vi "Launch Autocomplete Handler.vi"(4 "Shared Options (Local)":refnum<class "Shared Options.lvclass">, 5 "Autohide ListBox (F)":bool, 6 "Allow Undefined Values (F)":bool, 7 "ListBox Refnum (Popup)":refnum<vi>, 8 "error in (no error)":errorcluster, 9 "Height (200)":i16=200, 10 "Initial Options (Empty)":string[](array[string]), 11 "Str Refnum":refnum<vi>) -> (0 "error out":errorcluster, 1 "New Options Event":refnum<user-event>, 2 "Stop Event":refnum<user-event>, 3 "Selection":refnum<user-event>)   [LabVIEW 2020, in "AutoComplete.lvlib"]
doc: "Creates a standalone AutoComplete handler with separate events for interaction. Register for the <b>Selection</b> event to receive selections made by users with autocomplete. <b>Stop</b> and <b>New Options</b> events are for interacting to the autocomplete handler.\n\n<b>Str Refnum</b> - The control that drives the search functionality and has the result placed in.\n<b>Initial Options</b> - The starting list of possible selections. This can bae updated later by generating a New Options event.\n<b>Height</b> - Sets the pixel height of the popup list when typing into the specified string.\n<b>ListBox Refnum</b> - Alternatively a separate ListBox can be specified that is integrated into the UI.\n<b>Autohide ListBox</b> - When specifying an external ListBox, this causes the listbox to be hidden whenever a selection is made.\n<b>Allow Undefined Values</b> - Allows users to enter arbitrary values in addition to what is available in the options list.\n<b>Shared Options</b> - Uses the Shared Options instance, if valid, to filter available options from. If a Shared Options instance is specified, the Selection event output will not be available for use."
uses:
  AutoComplete.lvlib
  Shared Options/Shared Options.lvclass
  Shared Options/Shared Options.lvclass/Shared Options.ctl
  f473066a-8c46-4ba7-8d54-d92ea80dbf8d.vi/ff40df25-0e41-4205-825d-56c19dc320b6.vi
  <vilib>/Utility/Debug Log/Display.vi
  Autocomplete UI.vi
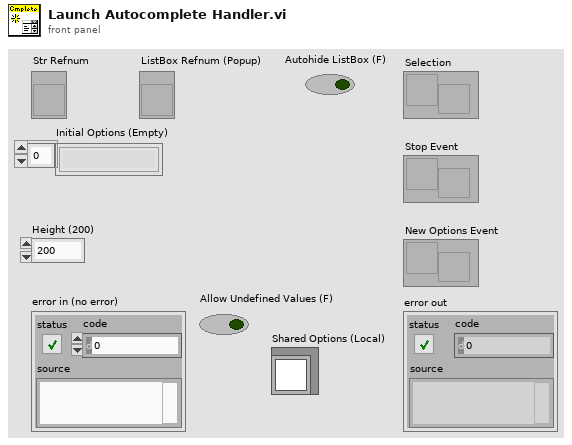
[diagram p1: front panel]
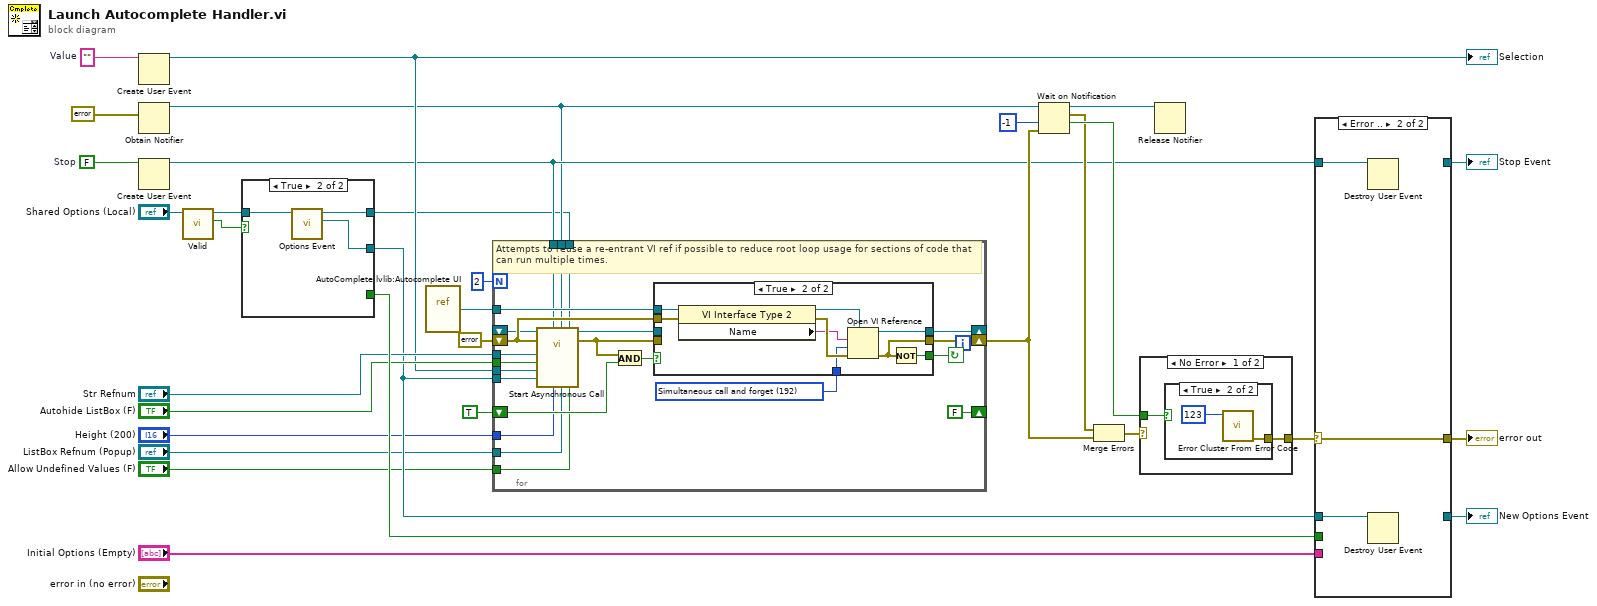
[diagram p0: block diagram]
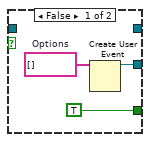
[diagram p3: hidden frame]
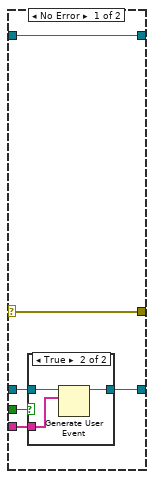
[diagram p6: hidden frame]
diagram:
  w20 = ""  # Value
  w32 = FALSE  # Stop
  n1 = Create User Event(user event datatype=w20) -> (user event=w9:refnum<user-event>)  [unwired: 1 in, 1 out]
  "Selection" <- w9
  n2 = Obtain Notifier(notification data type=errorcluster {"status"=FALSE, "code"=0, "source"=""} ("error constant")) -> (notifier out=w3:refnum<notifier>)  [unwired: 3 in, 2 out]
  n3 = Create User Event(user event datatype=w32) -> (user event=w4:refnum<user-event>)  [unwired: 1 in, 1 out]
  n4 = call "Valid.vi"("Shared Options in"="Shared Options (Local)") -> ("Valid"=w18:bool, "Shared Options out"=w17:refnum<class "Shared Options.lvclass">)  [unwired: 8 in, 1 out]
  n5 = case shown="True" w18 {
    tunnel: w17 -> [_ w38]
    tunnel: [w34 w36] -> w8
    tunnel: [_ w37] -> w2
    tunnel: [TRUE _] -> w16
    frame False {
      w35 = string[] []  # Options
      n6 = Create User Event(user event datatype=w35) -> (user event=w34:refnum<user-event>)  [unwired: 1 in, 1 out]
    }
    frame True {
      n7 = call "Options Event.vi"("Shared Options in"=w38) -> ("Options Event"=w36:refnum<user-event>, "Shared Options out"=w37:refnum<class "Shared Options.lvclass">)  [unwired: 8 in, 1 out]
    }
  }
  n8 = vi-ref "AutoComplete.lvlib:Autocomplete UI.vi"() -> (w14:refnum<vi>)
  n9 = for {
    N: 2 -> [_]
    tunnel: w14 -> [w59]
    shift-right: [w58] -> _
    shift-left: _ -> [w57]
    shift-right: [w55] -> w12
    shift-left: errorcluster {"status"=FALSE, "code"=0, "source"=""} ("error out") -> [w60]
    shift-right: [FALSE] -> _
    shift-left: TRUE -> [w52]
    tunnel: "Str Refnum" -> [w48]
    tunnel: "Autohide ListBox (F)" -> [w47]
    tunnel: w9 -> [w46]
    tunnel: w8 -> [w45]
    tunnel: "Height (200)" -> [w44]
    tunnel: "ListBox Refnum (Popup)" -> [w43]
    tunnel: "Allow Undefined Values (F)" -> [w42]
    tunnel: w4 -> [w41]
    tunnel: w3 -> [w40]
    tunnel: w2 -> [w39]
    stop <- w51 continue-if-true
    w49 = 192 items=["Record modifications"=1, "Open templates for editing"=2, "Prompt user to save"=4, "Prepare for reentrant run"=8, "Prompt to find missing subVIs"=16, "Hide loading dialog box"=32, "Enable simultaneous calls"=64, "Prepare to call and forget"=128, "Simultaneous call and forget"=192, "Prepare to call and collect"=256, "Simultaneous call and collect"=320]
    # "Attempts to reuse a re-entrant VI ref if possible to reduce root loop usage for sections of code that can run multiple times."
    n10 = call-by-ref "Start Asynchronous Call"(reference=w57, error in=w60, "Allow Undefined Values? (F)"=w42, "Shared Options (Local)"=w39, "LstBox Refnum"=w43, "Ready Notifier"=w40, "Height (200)"=w44, "Stop Event"=w41, "Options"=w45, "Selection Event"=w46, "Autohide ListBox (F)"=w47, "Str Refnum"=w48) -> (reference out=w56:refnum<vi>, error out=w54:errorcluster)  [unwired: 2 in]
    n11 = And(x=w54, y=w52) -> (x .and. y?=w53:bool)
    n12 = case shown="True" w53 {
      tunnel: w59 -> [_ w70]
      tunnel: w49 -> [_ w68]
      tunnel: [w62 w66] -> w58
      tunnel: w56 -> [w62 _]
      tunnel: [w61 w64] -> w55
      tunnel: w54 -> [w61 _]
      tunnel: w60 -> [_ w65]
      tunnel: [_ w63] -> w51
      frame False {
      }
      frame True {
        n13 = property class="VI Interface Type 2"(reference=w70, error in=w65) -> (reference out=w67:refnum<vi>, error out=w71:errorcluster, "Name"=w69:string)
        n14 = Open VI Reference(type specifier VI Refnum (for type only)=w67, vi path=w69, options=w68, error in (no error)=w71) -> (vi reference=w66:refnum<vi>, error out=w64:errorcluster)  [unwired: 2 in]
        n15 = Not(x=w64) -> (.not. x?=w63:bool)
      }
    }
  }
  n16 = Wait on Notification(notifier=w3, timeout in ms (-1)=-1, error in (no error)=w12) -> (notifier out=w29:refnum<notifier>, notification=w22:errorcluster, timed out?=w28:bool)  [unwired: 1 in, 1 out]
  n17 = Merge Errors(w22, w12) -> (w21:errorcluster)
  n18 = case shown="No Error" w21 {
    selector: w21 -> [_ w76]
    tunnel: w28 -> [w73 _]
    tunnel: [w72 w76] -> w27
    frame No Error {
      n19 = case shown="True" w73 {
        tunnel: [_ w74] -> w72
        frame False {
        }
        frame True {
          n20 = call <vilib>:"Error Cluster From Error Code.vi"("error code (0)"=123) -> ("error out"=w74:errorcluster)  [unwired: 8 in]
        }
      }
    }
    frame Error {
    }
  }
  n21 = Release Notifier(notifier=w29) -> ()  [unwired: 2 in, 3 out]
  n22 = case shown="Error .." w27 {
    selector: w27 -> [w81 w86]
    tunnel: w8 -> [w80 w87]
    tunnel: [w82 _] -> w26
    tunnel: w4 -> [w82 w88]
    tunnel: [w78 _] -> w25
    tunnel: [w81 w86] -> w24
    tunnel: "Initial Options (Empty)" -> [w79 _]
    tunnel: w16 -> [w77 _]
    frame No Error {
      n23 = case shown="True" w77 {
        tunnel: w80 -> [_ w85]
        tunnel: w79 -> [_ w84]
        tunnel: [_ w83] -> w78
        frame False {
        }
        frame True {
          n24 = Generate User Event(user event=w85, event data cluster=w84) -> (user event out=w83:refnum<user-event>)  [unwired: 2 in, 1 out]
        }
      }
    }
    frame Error {
      n25 = Destroy User Event(user event=w88) -> ()  [unwired: 1 in, 1 out]
      n26 = Destroy User Event(user event=w87) -> ()  [unwired: 1 in, 1 out]
    }
  }
  "Stop Event" <- w26
  "New Options Event" <- w25
  "error out" <- w24
